vi "user32 SetWindowLongPtrW.vi"(0 "hWnd":u64, 5 "nIndex":i32=-20, 7 "dwNewLong":i64, 11 "error in":errorcluster) -> (4 "return value":i64, 15 "error out":errorcluster)   [LabVIEW 2020, in "RemoteVI.lvlib"]
doc: "Writes a value of the window hWnd through user32.dll SetWindowLongPtrW (stdcall, called in any thread). nIndex -16 GWL_STYLE sets the window style, -20 GWL_EXSTYLE the extended style (WS_EX_LAYERED 0x80000). return value is the previous value; 0 can mean failure. When error in carries an error the DLL is not called. Generated by scripts\\Build Win32 Wrappers.vi - do not edit by hand, rebuild it."
uses:
  RemoteVI.lvlib
  user32.dll
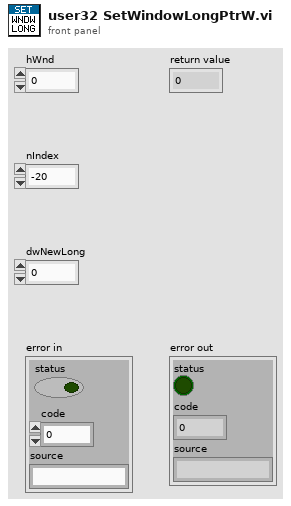
[diagram p1: front panel]
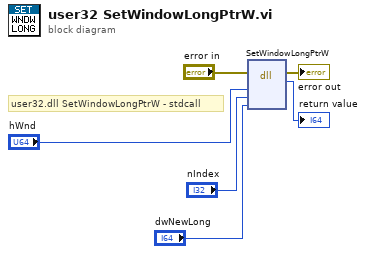
[diagram p0: block diagram]
diagram:
  # "user32.dll SetWindowLongPtrW - stdcall"
  n1 = dll-call lib="user32.dll" fn="SetWindowLongPtrW"(error in="error in", "hWnd"="hWnd", "nIndex"="nIndex", "dwNewLong"="dwNewLong") -> (error out=→"error out":errorcluster, →"return value":i64)  [unwired: 5 in, 1 out]
